vi "NEVSTOP-3rdParty-Dependencies_Post-Install Custom Action.vi"(10 "Variant":variant) -> (0 "error out":errorcluster)   [LabVIEW 2014]
uses:
  <vilib>/Palette API/Palette Menu/Public Type Define/Palette type.ctl
  <vilib>/Palette API/Palette Menu/Palette Menu.lvlib
panel:
  out "Array":path[](array[path])
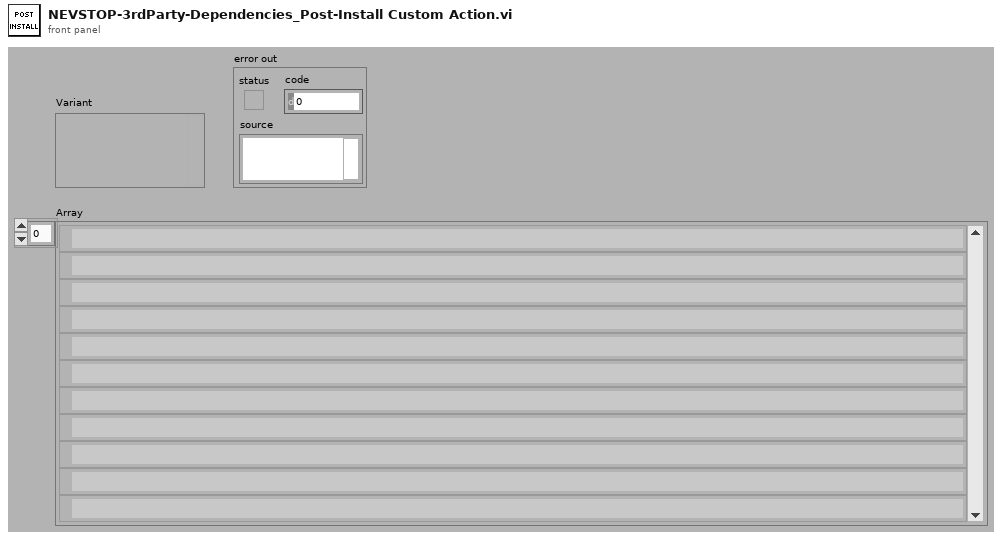
[diagram p1: front panel]
types:
  T1 = typedef "Palette Menu.lvlib/Palette type.ctl" = i32
  T2 = typedef "Palette Menu.lvlib/Palette Data.ctl" = cluster{"display name":string, "view format":T3, "palette width":i16, "items":T4, "256 color icon":picture, "B&W color icon":picture, "help information":T6, "palette description":string, "synchronize information":T7}
  T3 = typedef "Palette Menu.lvlib/View Format.ctl" = u16
  T4 = typedef "Palette Menu.lvlib/Items.ctl" = T5[]
  T5 = typedef "Palette Menu.lvlib/Item.ctl" = cluster{"item path":path, "library path (.lvlib)":path, "use default lvlib palette":bool, "short name":string, "place VI contents":bool, "hide synchronized item":bool, "reserve spot for synch item":bool, "configure when placing VI contents":bool}
  T6 = typedef "Palette Menu.lvlib/Help Info.ctl" = cluster{"help tag":string, "help file path ":path}
  T7 = typedef "Palette Menu.lvlib/Synchronize Info.ctl" = cluster{"synchronize with directory":bool, "synchronize directory path":path}
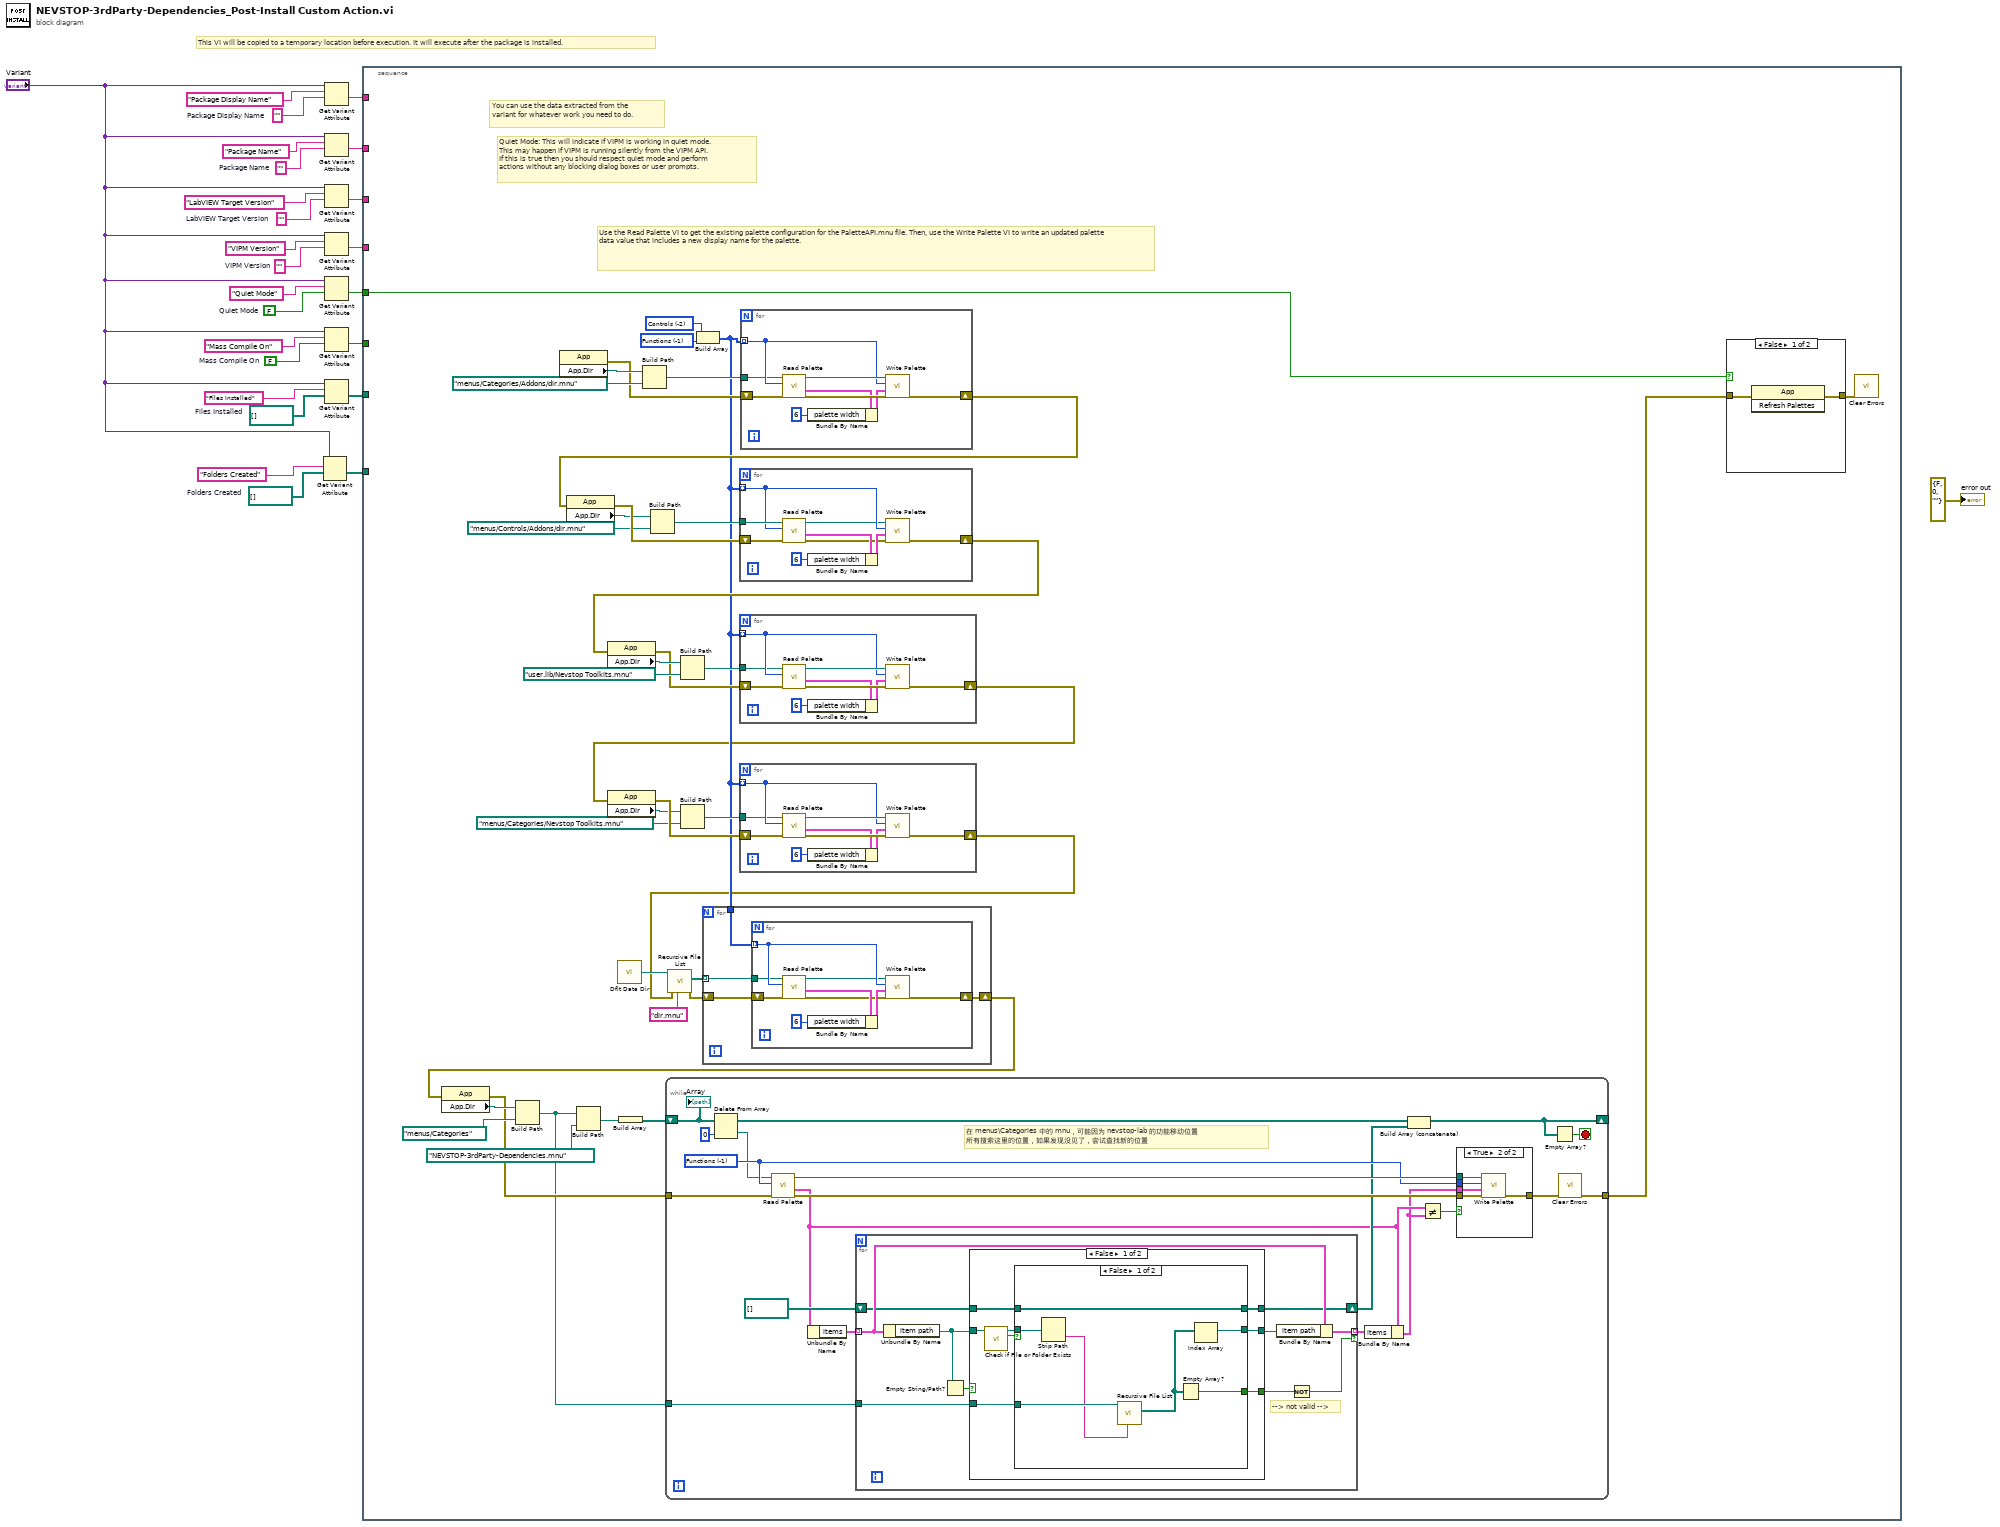
[diagram p0: block diagram]
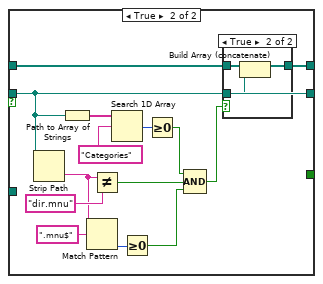
[diagram p3: hidden frame]
diagram:
  w1 = path[] []  # Folders Created
  w2 = path[] []  # Files Installed
  w8 = FALSE  # Mass Compile On
  w9 = ""  # Package Display Name
  w16 = FALSE  # Quiet Mode
  w19 = ""  # VIPM Version
  w21 = ""  # LabVIEW Target Version
  w23 = ""  # Package Name
  # "This VI will be copied to a temporary location before execution. It will execute after the package is installed."
  n1 = Get Variant Attribute(Variant="Variant", name="Folders Created", default value (empty Variant)=w1) -> (value=w6:path[])  [unwired: 1 in, 3 out]
  n2 = Get Variant Attribute(Variant="Variant", name="Package Display Name", default value (empty Variant)=w9) -> (value=w15:string)  [unwired: 1 in, 3 out]
  n3 = Get Variant Attribute(Variant="Variant", name="Package Name", default value (empty Variant)=w23) -> (value=w14:string)  [unwired: 1 in, 3 out]
  n4 = Get Variant Attribute(Variant="Variant", name="LabVIEW Target Version", default value (empty Variant)=w21) -> (value=w13:string)  [unwired: 1 in, 3 out]
  n5 = Get Variant Attribute(Variant="Variant", name="VIPM Version", default value (empty Variant)=w19) -> (value=w12:string)  [unwired: 1 in, 3 out]
  n6 = Get Variant Attribute(Variant="Variant", name="Quiet Mode", default value (empty Variant)=w16) -> (value=w11:bool)  [unwired: 1 in, 3 out]
  n7 = Get Variant Attribute(Variant="Variant", name="Mass Compile On", default value (empty Variant)=w8) -> (value=w10:bool)  [unwired: 1 in, 3 out]
  n8 = Get Variant Attribute(Variant="Variant", name="Files Installed", default value (empty Variant)=w2) -> (value=w5:path[])  [unwired: 1 in, 3 out]
  n9 = stacked-sequence {
    tunnel: w15 -> [_]
    tunnel: w14 -> [_]
    tunnel: w13 -> [_]
    tunnel: w12 -> [_]
    tunnel: w11 -> [w53]
    tunnel: w10 -> [_]
    tunnel: w5 -> [_]
    tunnel: w6 -> [_]
    frame #0 {
      w43 = T1 -2 items=["Functions"=-1, "Controls"=-2] ("palette type")
      w63 = T1 -1 items=["Functions"=-1, "Controls"=-2] ("palette type")
      # "Use the Read Palette VI to get the existing palette configuration for the PaletteAPI.mnu file. Then, use the Write Palette VI to write an updated palette data value that includes a new display name for the palette."
      # "Quiet Mode: This will indicate if VIPM is working in quiet mode.\nThis may happen if VIPM is running silently from the VIPM API.\nIf this is true then you should respect quiet mode and perform\nactions without any blocking dialog boxes or user prompts."
      # "You can use the data extracted from the variant for whatever work you need to do."
      n10 = property class="App"() -> (error out=w59:errorcluster, "App.Dir"=w62:path)  [unwired: 2 in, 1 out]
      n11 = call <vilib>:"Dflt Data Dir.vi"() -> ("App:Default Data Directory"=w52:path)
      n12 = Build Path(base path=w62, name or relative path=path "menus/Categories/Addons/dir.mnu") -> (appended path=w61:path)
      n13 = Build Array(w43, w63) -> (w38:T1[])
      n14 = for {
        tunnel: w38 -> [w167] mode=indexing
        tunnel: w61 -> [w166]
        shift-right: [w163] -> w54
        shift-left: w59 -> [w165]
        n15 = call <vilib>:"Read Palette.vi"("error in (no error)"=w165, "palette type"=w167, "palette path"=w166) -> ("error out"=w171:errorcluster, "palette data"=w170:T2, "duplicate palette path"=w168:path)  [unwired: 1 in, 5 out]
        n16 = Bundle By Name(cluster=w170, "palette width"=i16 6) -> (w169:T2)
        n17 = call <vilib>:"Write Palette.vi"("error in (no error)"=w171, "palette data"=w169, "palette type"=w167, "palette path"=w168) -> ("error out"=w163:errorcluster)  [unwired: 1 in, 6 out]
      }
      n18 = property class="App"(error in=w54) -> (error out=w58:errorcluster, "App.Dir"=w55:path)  [unwired: 1 in, 1 out]
      n19 = Build Path(base path=w55, name or relative path=path "menus/Controls/Addons/dir.mnu") -> (appended path=w56:path)
      n20 = for {
        tunnel: w56 -> [w160]
        tunnel: w38 -> [w159] mode=indexing
        shift-right: [w154] -> w44
        shift-left: w58 -> [w161]
        n21 = call <vilib>:"Read Palette.vi"("error in (no error)"=w161, "palette type"=w159, "palette path"=w160) -> ("error out"=w155:errorcluster, "palette data"=w156:T2, "duplicate palette path"=w158:path)  [unwired: 1 in, 5 out]
        n22 = Bundle By Name(cluster=w156, "palette width"=i16 6) -> (w157:T2)
        n23 = call <vilib>:"Write Palette.vi"("error in (no error)"=w155, "palette data"=w157, "palette type"=w159, "palette path"=w158) -> ("error out"=w154:errorcluster)  [unwired: 1 in, 6 out]
      }
      n24 = property class="App"(error in=w44) -> (error out=w45:errorcluster, "App.Dir"=w48:path)  [unwired: 1 in, 1 out]
      n25 = Build Path(base path=w48, name or relative path=path "user.lib/Nevstop Toolkits.mnu") -> (appended path=w47:path)
      n26 = for {
        tunnel: w38 -> [w149] mode=indexing
        tunnel: w47 -> [w148]
        shift-right: [w145] -> w37
        shift-left: w45 -> [w147]
        n27 = call <vilib>:"Read Palette.vi"("error in (no error)"=w147, "palette type"=w149, "palette path"=w148) -> ("error out"=w153:errorcluster, "palette data"=w152:T2, "duplicate palette path"=w150:path)  [unwired: 1 in, 5 out]
        n28 = Bundle By Name(cluster=w152, "palette width"=i16 6) -> (w151:T2)
        n29 = call <vilib>:"Write Palette.vi"("error in (no error)"=w153, "palette data"=w151, "palette type"=w149, "palette path"=w150) -> ("error out"=w145:errorcluster)  [unwired: 1 in, 6 out]
      }
      n30 = property class="App"(error in=w37) -> (error out=w42:errorcluster, "App.Dir"=w39:path)  [unwired: 1 in, 1 out]
      n31 = Build Path(base path=w39, name or relative path=path "menus/Categories/Nevstop Toolkits.mnu") -> (appended path=w40:path)
      n32 = for {
        tunnel: w38 -> [w140] mode=indexing
        tunnel: w40 -> [w139]
        shift-right: [w136] -> w36
        shift-left: w42 -> [w138]
        n33 = call <vilib>:"Read Palette.vi"("error in (no error)"=w138, "palette type"=w140, "palette path"=w139) -> ("error out"=w144:errorcluster, "palette data"=w143:T2, "duplicate palette path"=w141:path)  [unwired: 1 in, 5 out]
        n34 = Bundle By Name(cluster=w143, "palette width"=i16 6) -> (w142:T2)
        n35 = call <vilib>:"Write Palette.vi"("error in (no error)"=w144, "palette data"=w142, "palette type"=w140, "palette path"=w141) -> ("error out"=w136:errorcluster)  [unwired: 1 in, 6 out]
      }
      n36 = call <vilib>:"Recursive File List.vi"("pattern"="dir.mnu", "error in (no error)"=w36, "Folder Path"=w52) -> ("error out"=w49:errorcluster, "All Files in Dir"=w50:path[])  [unwired: 4 in, 3 out]
      n37 = for {
        tunnel: w50 -> [w175] mode=indexing
        shift-right: [w173] -> w32
        shift-left: w49 -> [w174]
        tunnel: w38 -> [w172]
        n38 = for {
          tunnel: w172 -> [w183] mode=indexing
          tunnel: w175 -> [w178]
          shift-right: [w176] -> w173
          shift-left: w174 -> [w177]
          n39 = call <vilib>:"Read Palette.vi"("error in (no error)"=w177, "palette type"=w183, "palette path"=w178) -> ("error out"=w179:errorcluster, "palette data"=w180:T2, "duplicate palette path"=w182:path)  [unwired: 1 in, 5 out]
          n40 = Bundle By Name(cluster=w180, "palette width"=i16 6) -> (w181:T2)
          n41 = call <vilib>:"Write Palette.vi"("error in (no error)"=w179, "palette data"=w181, "palette type"=w183, "palette path"=w182) -> ("error out"=w176:errorcluster)  [unwired: 1 in, 6 out]
        }
      }
      n42 = property class="App"(error in=w32) -> (error out=w33:errorcluster, "App.Dir"=w35:path)  [unwired: 1 in, 1 out]
      n43 = Build Path(base path=w35, name or relative path=path "menus/Categories") -> (appended path=w30:path)
      n44 = Build Path(base path=w30, name or relative path=path "NEVSTOP-3rdParty-Dependencies.mnu") -> (appended path=w29:path)
      n45 = Build Array(w29) -> (w31:path[])
      n46 = while {
        tunnel: w33 -> [w84]
        shift-right: [w71] -> _
        shift-left: w31 -> [w76]
        tunnel: w30 -> [w78]
        tunnel: [w69] -> w27
        stop <- w74 stop-if-true
        w79 = T1 -1 items=["Functions"=-1, "Controls"=-2] ("palette type")
        # "在 menus\\Categories 中的 mnu，可能因为 nevstop-lab 的功能移动位置\n所有搜索这里的位置，如果发现没见了，尝试查找新的位置"
        n47 = Delete From Array(array=w76, index=0) -> (deleted portion=w77:path, array with subset deleted=w73:path[])  [unwired: 1 in]
        n48 = call <vilib>:"Read Palette.vi"("error in (no error)"=w84, "palette type"=w79, "palette path"=w77) -> ("error out"=w83:errorcluster, "palette data"=w67:T2, "duplicate palette path"=w82:path)  [unwired: 1 in, 5 out]
        n49 = Unbundle By Name(w67) -> ("items"=w81:T4)
        n50 = for {
          tunnel: w81 -> [w100] mode=indexing
          tunnel: [w98] -> w80 mode=indexing if=w95
          tunnel: w78 -> [w97]
          shift-right: [w93] -> w70
          shift-left: path[] [] -> [w94]
          # "--> not valid -->"
          n51 = Unbundle By Name(w100) -> ("item path"=w91:path)
          n52 = Empty String/Path?(string/path=w91) -> (empty?=w92:bool)
          n53 = case shown="False" w92 {
            tunnel: w91 -> [w107 w135]
            tunnel: [w104 w135] -> w99
            tunnel: w97 -> [w108 _]
            tunnel: [w103 _] -> w96
            tunnel: w94 -> [w101 w134]
            tunnel: [w102 w134] -> w93
            frame False {
              n54 = call <vilib>:"Check if File or Folder Exists.vi"("path"=w107) -> ("file or folder exists?"=w106:bool, "dup path"=w105:path)  [unwired: 8 in, 1 out]
              n55 = case shown="False" w106 {
                tunnel: w108 -> [w115 _]
                tunnel: w105 -> [w110 w118]
                tunnel: [w114 w118] -> w104
                tunnel: [w112 _] -> w103
                tunnel: [w111 w128] -> w102
                tunnel: w101 -> [w111 w129]
                frame False {
                  n56 = Strip Path(path=w110) -> (name=w109:string)  [unwired: 1 out]
                  n57 = call <vilib>:"Recursive File List.vi"("pattern"=w109, "Folder Path"=w115) -> ("All Files in Dir"=w113:path[])  [unwired: 5 in, 4 out]
                  n58 = Empty Array?(array=w113) -> (empty?=w112:bool)
                  n59 = Index Array(array=w113) -> (element=w114:path)  [unwired: 1 in]
                }
                frame True {
                  n60 = Strip Path(path=w118) -> (name=w125:string)  [unwired: 1 out]
                  n61 = Path to Array of Strings(0:w118) -> (2:w119:string[])  [unwired: 1 out]
                  n62 = Match Pattern(string=w125, regular expression=".mnu$") -> (offset past match=w123:i32)  [unwired: 1 in, 3 out]
                  n63 = Not Equal?(x=w125, y="dir.mnu") -> (x != y?=w127:bool)
                  n64 = Search 1D Array(1D array=w119, element="Categories") -> (index of element=w117:i32)  [unwired: 1 in]
                  n65 = Greater Or Equal To 0?(x=w123) -> (x >= 0?=w122:bool)
                  n66 = Greater Or Equal To 0?(x=w117) -> (x >= 0?=w116:bool)
                  n67 = Compound Arithmetic op=AND(w116, w127, w122) -> (w121:bool)
                  n68 = case shown="True" w121 {
                    tunnel: w129 -> [w130 w133]
                    tunnel: [w130 w132] -> w128
                    tunnel: w118 -> [_ w131]
                    frame False {
                    }
                    frame True {
                      n69 = Build Array (concatenate)(w133, w131) -> (w132:path[])
                    }
                  }
                }
              }
            }
            frame True {
            }
          }
          n70 = Bundle By Name(cluster=w100, "item path"=w99) -> (w98:T5)
          n71 = Not(x=w96) -> (.not. x?=w95:bool)
        }
        n72 = Bundle By Name(cluster=w67, "items"=w80) -> (w66:T2)
        n73 = Build Array (concatenate)(w73, w70) -> (w71:path[])
        n74 = Not Equal?(x=w67, y=w66) -> (x != y?=w65:bool)
        n75 = case shown="True" w65 {
          tunnel: w83 -> [w85 w90]
          tunnel: w82 -> [_ w89]
          tunnel: w79 -> [_ w88]
          tunnel: [w85 w87] -> w68
          tunnel: w66 -> [_ w86]
          frame False {
          }
          frame True {
            n76 = call <vilib>:"Write Palette.vi"("error in (no error)"=w90, "palette data"=w86, "palette type"=w88, "palette path"=w89) -> ("error out"=w87:errorcluster)  [unwired: 1 in, 6 out]
          }
        }
        n77 = Empty Array?(array=w71) -> (empty?=w74:bool)
        n78 = call <vilib>:"Clear Errors.vi"("error in (no error)"=w68) -> ("error out"=w69:errorcluster)  [unwired: 6 in]
        "Array" <- w76
      }
      n79 = case shown="False" w53 {
        tunnel: [w186 w187] -> w64
        tunnel: w27 -> [w185 w187]
        frame False {
          n80 = invoke class="App" method="Refresh Palettes"(error in=w185) -> (error out=w186:errorcluster)  [unwired: 2 in, 2 out]
        }
        frame True {
        }
      }
      n81 = call <vilib>:"Clear Errors.vi"("error in (no error)"=w64) -> ()  [unwired: 6 in, 1 out]
    }
  }
  "error out" <- errorcluster {"status"=FALSE, "code"=0, "source"=""} ("error out")
